vi "_AddOverlayGroup.vi"(8 "error in":errorcluster, 10 "GroupName":string, 11 "Image Reference In":T1) -> (0 "error out":errorcluster, 3 "Image Reference Out":T1)   [LabVIEW 2020, in "OpenLvVision_Overlays.lvlib"]
uses:
  OpenLvVision_Overlays.lvlib
  <vilib>/OpenLvVision/OpenLvVision_Image/Management/TypeDef/OLV Image.ctl
  <vilib>/OpenLvVision/OpenLvVision_Image/Management/OLV Management.lvlib
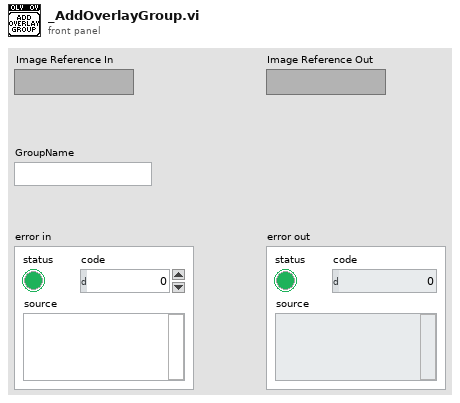
[diagram p1: front panel]
types:
  T1 = typedef "OLV OpenLvVision_Image.lvlib/OLV Management.lvlib/OLV Image.ctl" = refnum<image>
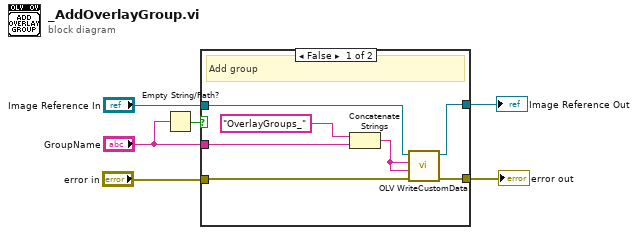
[diagram p0: block diagram]
diagram:
  n1 = Empty String/Path?(string/path="GroupName") -> (empty?=w1:bool)
  n2 = case shown="False" w1 {
    tunnel: "GroupName" -> [w12 _]
    tunnel: "Image Reference In" -> [w11 w15]
    tunnel: [w10 w15] -> w5
    tunnel: "error in" -> [w9 w14]
    tunnel: [w8 w14] -> w3
    frame False {
      # "Add group"
      n3 = Concatenate Strings("OverlayGroups_" ("string"), w12) -> (w7:string)
      n4 = call <vilib>:"OLV WriteCustomData.vi"("error in"=w9, "Data"=w7, "Key"=w7, "Image Reference In"=w11) -> ("error out"=w8:errorcluster, "Image Reference Out"=w10:T1)  [unwired: 6 in]
    }
    frame True {
      # "no group"
    }
  }
  "error out" <- w3
  "Image Reference Out" <- w5
